vi "draw.vi"(0 "reference in":refnum<class "VINode.lvclass">, 1 "graphics":refnum<class "Graphics.lvclass">, 5 "error in (no error)":errorcluster) -> (14 "reference out":refnum<class "VINode.lvclass">, 19 "error out":errorcluster)   [LabVIEW 2020, in "VINode.lvclass"]
doc: "public void draw(Graphics2D g2, Point2D p, Point2D q)"
uses:
  <resource>/Framework/Providers/Open_GDS/UML/VINode_class/VINode.lvclass
  C:/Program Files (x86)/National Instruments/LabVIEW 2020/resource/Framework/Providers/Open_GDS/UML/RectangularNode_class/RectangularNode.lvclass
  <resource>/Framework/Providers/Open_GDS/UML/Graphics_class/Graphics.lvclass
  <resource>/Framework/Providers/Open_GDS/UML/General/Rectangle/Rectangle Rectangle2D.ctl
  <resource>/Framework/Providers/Open_GDS/UML/UMLEditor/UMLEditor_StoredColors.ctl
  <resource>/Framework/Providers/Open_GDS/UML/MultiLineString_class/MultiLineString.lvclass
  <resource>/Framework/Providers/Open_GDS/UML/RectangularNode_class/RectangularNode.lvclass
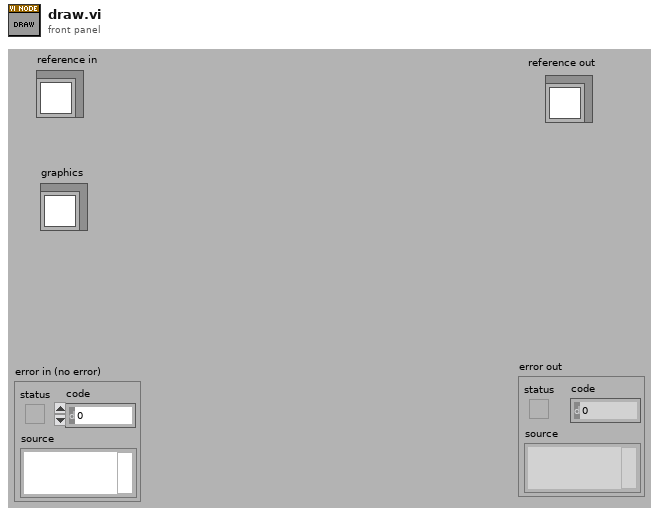
[diagram p1: front panel]
types:
  T1 = typedef "UMLEditor_StoredColors.ctl" = enum16{"ClassBackgroudColor", "ClassBackgroudColorWithClassPath", "ClassBackgroudColorForApplicationVIStereotype", "ClassBackgroudColorForTypeStereotype", "StateBackgroudColor", "ClassBackgroudColorForInterfaceStereotype"}
  T2 = typedef "Rectangle Rectangle2D.ctl" = cluster{"x":dbl, "y":dbl, "width":dbl, "height":dbl}
  T3 = typedef "VINode.lvclass/ObjectAttributes.ctl" = cluster{"midHeight":dbl, "botHeight":dbl, "Name":refnum<class "MultiLineString.lvclass">, "DEFAULT_COMPARTMENT_HEIGHT":i32, "DEFAULT_WIDTH":i32, "DEFAULT_HEIGHT":i32, "VIPath":path, "Description":refnum<class "MultiLineString.lvclass">, "ShowDescription":bool}
  T4 = typedef "RectangularNode.lvclass/ObjectAttributes.ctl" = cluster{"bounds":T2}
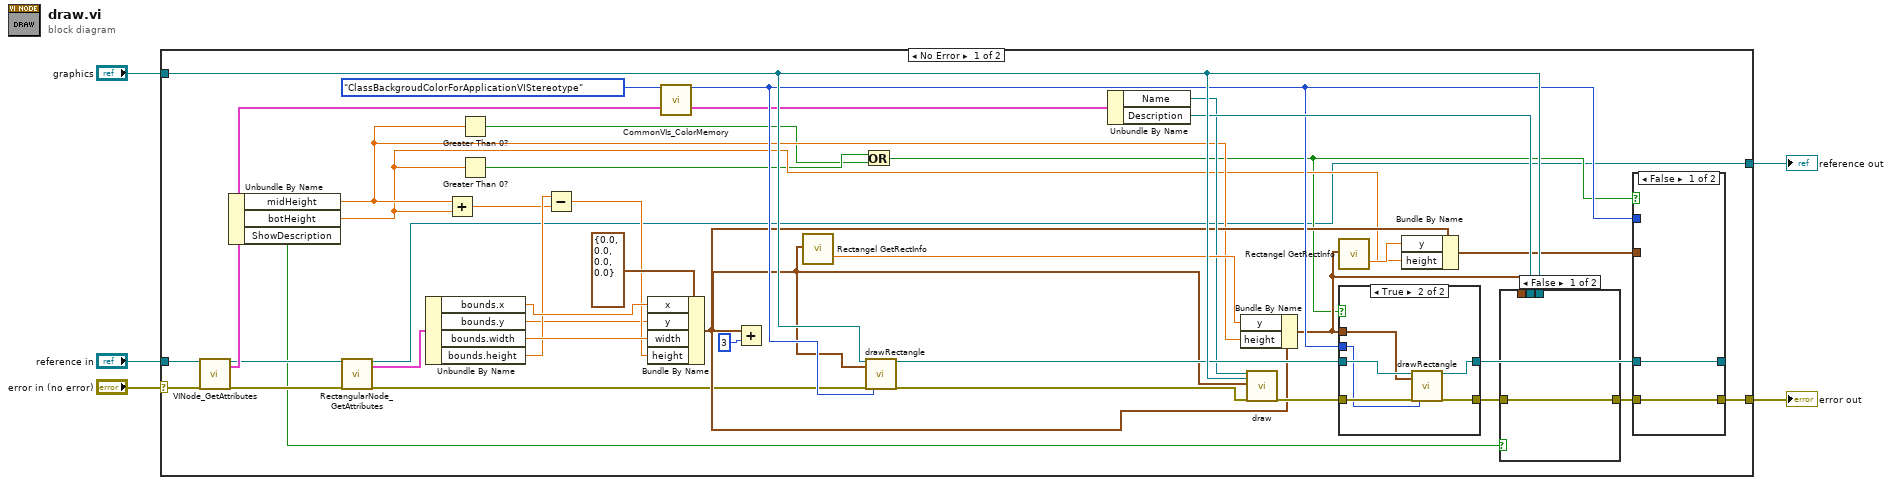
[diagram p0: block diagram]
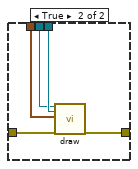
[diagram p2: hidden frame]
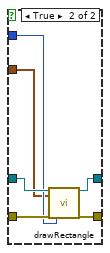
[diagram p3: hidden frame]
diagram:
  n1 = case shown="No Error" "error in (no error)" {
    selector: "error in (no error)" -> [w42 w67]
    tunnel: "reference in" -> [w44 w68]
    tunnel: [w7 w67] -> w4
    tunnel: [w10 w68] -> w3
    tunnel: "graphics" -> [w43 _]
    frame No Error {
      n2 = call <resource>:"VINode_GetAttributes.vi"("reference in"=w44, "error in (no error)"=w42) -> ("reference out"=w12:refnum<class "VINode.lvclass">, "Data"=w13:T3, "error out"=w11:errorcluster)  [unwired: 1 in, 14 out]
      n3 = Unbundle By Name(w13) -> ("midHeight"=w18:dbl, "botHeight"=w17:dbl, "ShowDescription"=w6:bool)
      n4 = call <resource>:"RectangularNode_GetAttributes.vi"("reference in"=w12, "error in (no error)"=w11) -> ("reference out"=w10:refnum<class "VINode.lvclass">, "Data"=w9:T4, "error out"=w8:errorcluster)  [unwired: 14 in, 1 out]
      n5 = Unbundle By Name(w9) -> ("bounds.x"=w40:dbl, "bounds.y"=w36:dbl, "bounds.width"=w39:dbl, "bounds.height"=w38:dbl)
      n6 = Add(x=w18, y=w17) -> (x+y=w35:dbl)
      n7 = Greater Than 0?(x=w18) -> (x > 0?=w15:bool)
      n8 = Greater Than 0?(x=w17) -> (x > 0?=w16:bool)
      n9 = Subtract(x=w38, y=w35) -> (x-y=w37:dbl)
      n10 = Bundle By Name(cluster=T2 {"x"=0.0, "y"=0.0, "width"=0.0, "height"=0.0} ("points"), "x"=w40, "y"=w36, "width"=w39, "height"=w37) -> (w20:T2)
      n11 = call <resource>:"CommonVIs_ColorMemory.vi"("ColorName"=UMLEditor_StoredColors."ClassBackgroudColorForApplicationVIStereotype" ("UMLPathes")) -> ("Color Out"=w24:u32)  [unwired: 3 in, 15 out]
      n12 = Add(x=w20, y=3) -> ()  [unwired: 1 out]
      n13 = call <resource>:"Rectangel GetRectInfo.vi"("bounds"=w20) -> ("maxY"=w27:dbl)  [unwired: 1 in, 17 out]
      n14 = Or(x=w16, y=w15) -> (x .or. y?=w14:bool)
      n15 = call <resource>:"drawRectangle.vi"("reference"=w43, "rectangle"=w20, "error in (no error)"=w8, "FillClor(if not used=BorderColorIsUsed,AutoFill)"=w24) -> ("reference out"=w34:refnum<class "Graphics.lvclass">, "error out"=w32:errorcluster)  [unwired: 3 in, 11 out]
      n16 = Unbundle By Name(w13) -> ("Name"=w25:refnum<class "MultiLineString.lvclass">, "Description"=w28:refnum<class "MultiLineString.lvclass">)
      n17 = Bundle By Name(cluster=w20, "y"=w27, "height"=w18) -> (w19:T2)
      n18 = call-dynamic "draw.vi"("reference"=w25, "graphics"=w43, "bounds"=w20, "error in (no error)"=w32) -> ("error out"=w31:errorcluster)  [unwired: 14 in, 1 out]
      n19 = call <resource>:"Rectangel GetRectInfo.vi"("bounds"=w19) -> ("maxY"=w26:dbl)  [unwired: 1 in, 17 out]
      n20 = case shown="True" w14 {
        tunnel: w34 -> [w60 w66]
        tunnel: [w60 w65] -> w33
        tunnel: w31 -> [w59 w64]
        tunnel: [w59 w63] -> w30
        tunnel: w24 -> [_ w62]
        tunnel: w19 -> [_ w61]
        frame False {
        }
        frame True {
          n21 = call <resource>:"drawRectangle.vi"("reference"=w66, "rectangle"=w61, "error in (no error)"=w64, "FillClor(if not used=BorderColorIsUsed,AutoFill)"=w62) -> ("reference out"=w65:refnum<class "Graphics.lvclass">, "error out"=w63:errorcluster)  [unwired: 3 in, 11 out]
        }
      }
      n22 = Bundle By Name(cluster=w20, "y"=w26, "height"=w17) -> (w22:T2)
      n23 = case shown="False" w6 {
        tunnel: w43 -> [_ w50]
        tunnel: w30 -> [w45 w49]
        tunnel: [w45 w48] -> w29
        tunnel: w28 -> [_ w47]
        tunnel: w19 -> [_ w46]
        frame False {
        }
        frame True {
          n24 = call-dynamic "draw.vi"("reference"=w47, "graphics"=w50, "bounds"=w46, "error in (no error)"=w49) -> ("error out"=w48:errorcluster)  [unwired: 14 in, 1 out]
        }
      }
      n25 = case shown="False" w14 {
        tunnel: w33 -> [w51 w58]
        tunnel: w29 -> [w52 w57]
        tunnel: [w52 w56] -> w7
        tunnel: w24 -> [_ w55]
        tunnel: w22 -> [_ w54]
        tunnel: [w51 w53] -> _
        frame False {
        }
        frame True {
          n26 = call <resource>:"drawRectangle.vi"("reference"=w58, "rectangle"=w54, "error in (no error)"=w57, "FillClor(if not used=BorderColorIsUsed,AutoFill)"=w55) -> ("reference out"=w53:refnum<class "Graphics.lvclass">, "error out"=w56:errorcluster)  [unwired: 3 in, 11 out]
        }
      }
    }
    frame Error {
    }
  }
  "reference out" <- w3
  "error out" <- w4
